vi "select_lane.vi"(4 "left":bool, 5 "right_line_edge":dbl, 6 "mid_roi_dead":bool, 7 "left_roi_dead":bool, 8 "mid_center in":dbl, 9 "rigt":bool, 10 "left_line_edge":dbl, 11 "right_roi_dead":bool) -> (2 "target_center":dbl, 3 "roi_reset":bool)   [LabVIEW 2024]
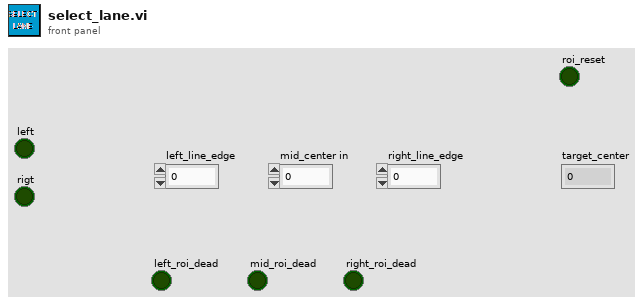
[diagram p1: front panel]
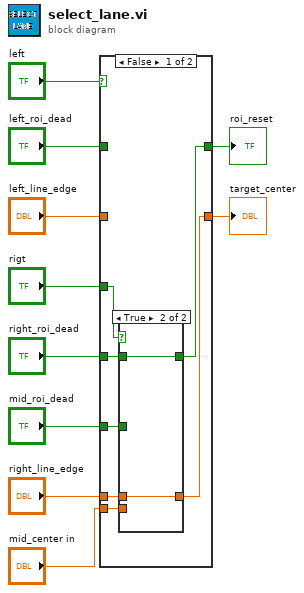
[diagram p0: block diagram]
diagram:
  n1 = case shown="False" "left" {
    tunnel: [w16 w23] -> w9
    tunnel: "left_line_edge" -> [_ w23]
    tunnel: [w15 w22] -> w10
    tunnel: "right_line_edge" -> [w17 _]
    tunnel: "left_roi_dead" -> [_ w22]
    tunnel: "rigt" -> [w14 _]
    tunnel: "right_roi_dead" -> [w13 _]
    tunnel: "mid_center in" -> [w12 _]
    tunnel: "mid_roi_dead" -> [w11 _]
    frame False {
      n2 = case shown="True" w14 {
        tunnel: [w19 w21] -> w16
        tunnel: w17 -> [_ w21]
        tunnel: [w18 w20] -> w15
        tunnel: w13 -> [_ w20]
        tunnel: w12 -> [w19 _]
        tunnel: w11 -> [w18 _]
        frame False {
        }
        frame True {
        }
      }
    }
    frame True {
    }
  }
  "roi_reset" <- w10
  "target_center" <- w9
